vi "AlliGator Set Special Phasor Frequency.vi"(8 "error in":errorcluster, 10 "ItemTag":string, 11 "Frequency Refnum":refnum<vi>) -> (0 "error out":errorcluster)   [LabVIEW 2021, in "AlliGator Phasor Graph.lvlib"]
uses:
  AlliGator Phasor Graph.lvlib
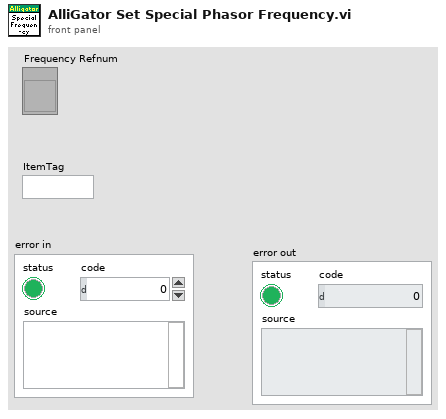
[diagram p1: front panel]
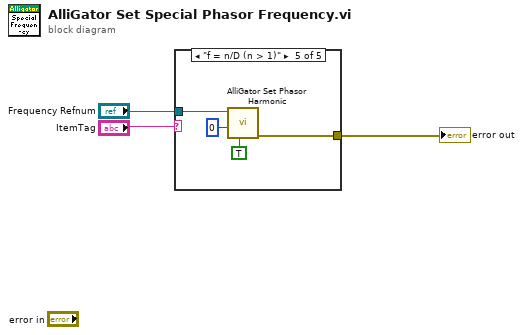
[diagram p0: block diagram]
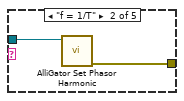
[diagram p3: hidden frame]
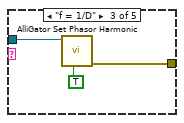
[diagram p4: hidden frame]
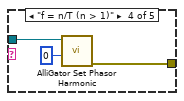
[diagram p5: hidden frame]
diagram:
  n1 = case shown="\"f = n/D (n > 1)\"" "ItemTag" {
    tunnel: "Frequency Refnum" -> [_ w5 w8 w11 w15]
    tunnel: [_ w4 w6 w9 w12] -> w3
    frame "", Default {
    }
    frame "f = 1/T" {
      n2 = call "AlliGator Set Phasor Harmonic.vi"("Phasor Frequency Refnum"=w5) -> ("Error Out"=w4:errorcluster)  [unwired: 10 in]
    }
    frame "f = 1/D" {
      n3 = call "AlliGator Set Phasor Harmonic.vi"("Use n/D"=TRUE, "Phasor Frequency Refnum"=w8) -> ("Error Out"=w6:errorcluster)  [unwired: 9 in]
    }
    frame "f = n/T (n > 1)" {
      n4 = call "AlliGator Set Phasor Harmonic.vi"("Harmonic (1)"=0, "Phasor Frequency Refnum"=w11) -> ("Error Out"=w9:errorcluster)  [unwired: 9 in]
    }
    frame "f = n/D (n > 1)" {
      n5 = call "AlliGator Set Phasor Harmonic.vi"("Use n/D"=TRUE, "Harmonic (1)"=0, "Phasor Frequency Refnum"=w15) -> ("Error Out"=w12:errorcluster)  [unwired: 8 in]
    }
  }
  "error out" <- w3
